vi "4Pi Astigmatism Alignment.vi"(7 "Calling VI Ref":refnum<vi>) -> ()   [LabVIEW 2016]
uses:
  <vilib>/Utility/miscctls.llb/LVPointTypeDef.ctl
  4Pi Astigmatism Alignment Type Defs/4Pi AA Notifier Type.ctl
  4Pi Astigmatism Alignment Type Defs/4Pi AA Actions.ctl
  <vilib>/vision/Image Controls.llb/IMAQ Image.ctl
  Hardware Configuration/Hardware Configuration Controls/Device Type.ctl
  Hardware Configuration/Hardware Configuration Controls/Device Function.ctl
  Device Library/Cameras/Hamamatsu/Orca Flash/Orca Flash Controls/Orca Flash Actions.ctl
  Device Library/Shutters/Shutter Controls/Shutter Actions.ctl
  Device Library/Stages/Stages Controls/Stage Actions.ctl
  <vilib>/Analysis/polynomials.llb/Polynomial Plot (Range).vi
  <vilib>/Analysis/NI_AALPro.lvlib
panel:
  out "Error":bool
  in  "Frame Accumulations":u16=1
  in  "Number of Steps":u16=10
  in  "Step Size (µm)":dbl=0.05
  in  "Scan and Align":bool
  in  "Scan Lower Obj":bool
  out "ROI Fit":dbl[][](graph)
  out "ROI Image":u16[][](graph)
  in  "Image Selection":i32(ring) items=["Quad 01", "Quad 02", "Quad 03", "Quad 04"]
  in  "Scan Upper Obj":bool
  in  "Quit":bool
  out "Scan Data":cluster{dbl[], dbl[]}[](graph)
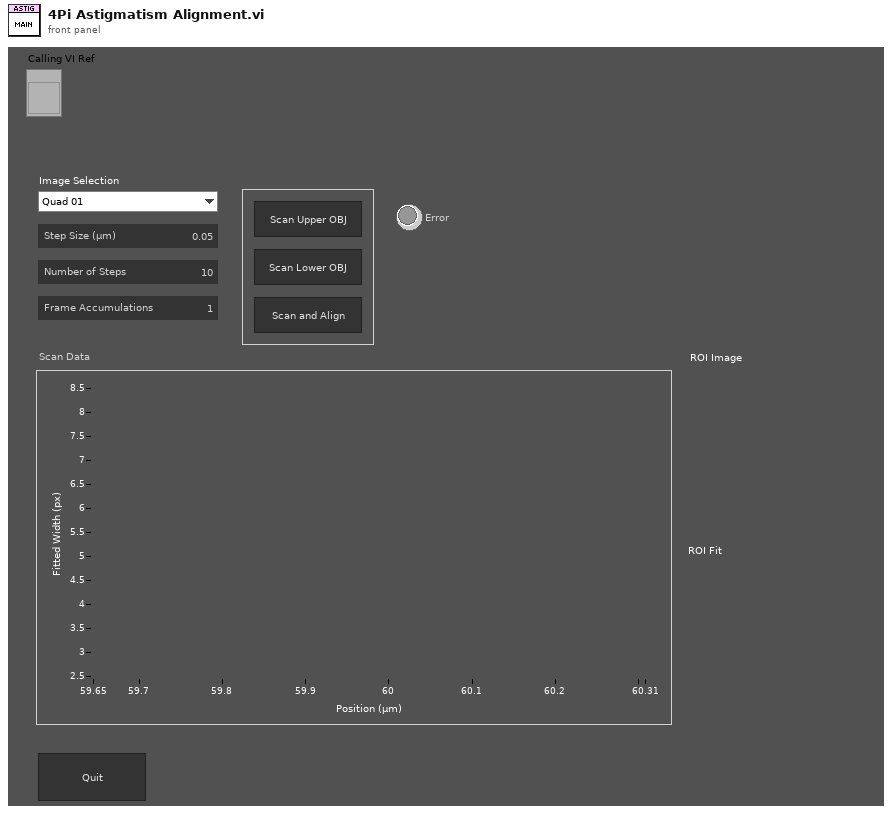
[diagram p1: front panel]
types:
  T1 = typedef "IMAQ Image.ctl" = refnum<image>
  T2 = typedef "4Pi AA Actions.ctl" = enum16{"Idle", "Scan Upper", "Scan Lower", "Scan and Align", "Open Shutter", "Close Shutter", "Set Z Start", "Get Image", "Plot Data", "Move Z Stage", "Fit Astig Curves", "Return Z Stage", "Switch", "Align OBJs", "Abort", "Quit"}
  T3 = typedef "4Pi AA Notifier Type.ctl" = cluster{"Actions":T2, "Scan Steps":u16, "Step Size (µm)":dbl, "Frame Accums":u16, "Image Ref":T1, "Initial Z Pos (µm)":dbl}
  T4 = enum16{"Always On", "Always Off", "Off While Running"}
  T5 = typedef "LVPointTypeDef.ctl" = cluster{"Horizontal":i16, "Vertical":i16}
  T6 = typedef "Device Function.ctl" = enum16{"Primary", "Secondary", "Overview", "Wide Field Drift Correction", "642 nm Excitation", "560 nm Excitation", "546 nm Excitation", "488 nm Excitation", "405 nm Excitation", "Objective Drift Correction", "Objective XY", "Objective Z", "Sample XY", "Sample Coarse Z", "Sample Z", "4Pi Lower", "4Pi Upper", "Adj Cavity", "Line Scanning", "Alert"}
  T7 = typedef "Device Type.ctl" = enum16{"AOTF", "Camera", "Deformable Mirror", "Laser", "Shutter", "Stage", "Waveform", "Email"}
  T8 = typedef "Orca Flash Actions.ctl" = enum16{"IDLE", "PREVIEW", "RECORD", "Record Settings", "SETPARAM", "GETPARAM", "SETROI", "GETROI", "PROGRESSIVE MODE", "AREA MODE", "STATUS", "QUIT"}
  T9 = typedef "Shutter Actions.ctl" = enum16{"Open", "Close", "Toggle", "Status", "Quit"}
  T10 = typedef "Stage Actions.ctl" = enum16{"Get Position", "MVR", "MOVE", "HALT", "ONTARGET", "ERROR", "REFERENCE", "INIT", "VELOCITY", "STATUS", "EXIT", "HOME", "ZEROPOS", "NANOPOS", "ANALOG", "QUIT"}
  T11 = enum32{"Invalid", "Standard", "Closed", "Hidden", "Minimized", "Maximized"}
  T12 = typedef "2D Gaussian - Best Fit Parameters.ctl" = cluster{"Amplitude":dbl, "X Position":dbl, "Y Position":dbl, "X Width":dbl, "Y Width":dbl, "Offset":dbl}
  T13 = typedef "LVRectTypeDef.ctl" = cluster{"Left":i16, "Top":i16, "Right":i16, "Bottom":i16}
  T14 = typedef "LVBoundsTypeDef.ctl" = cluster{"Width":u32, "Height":u32}
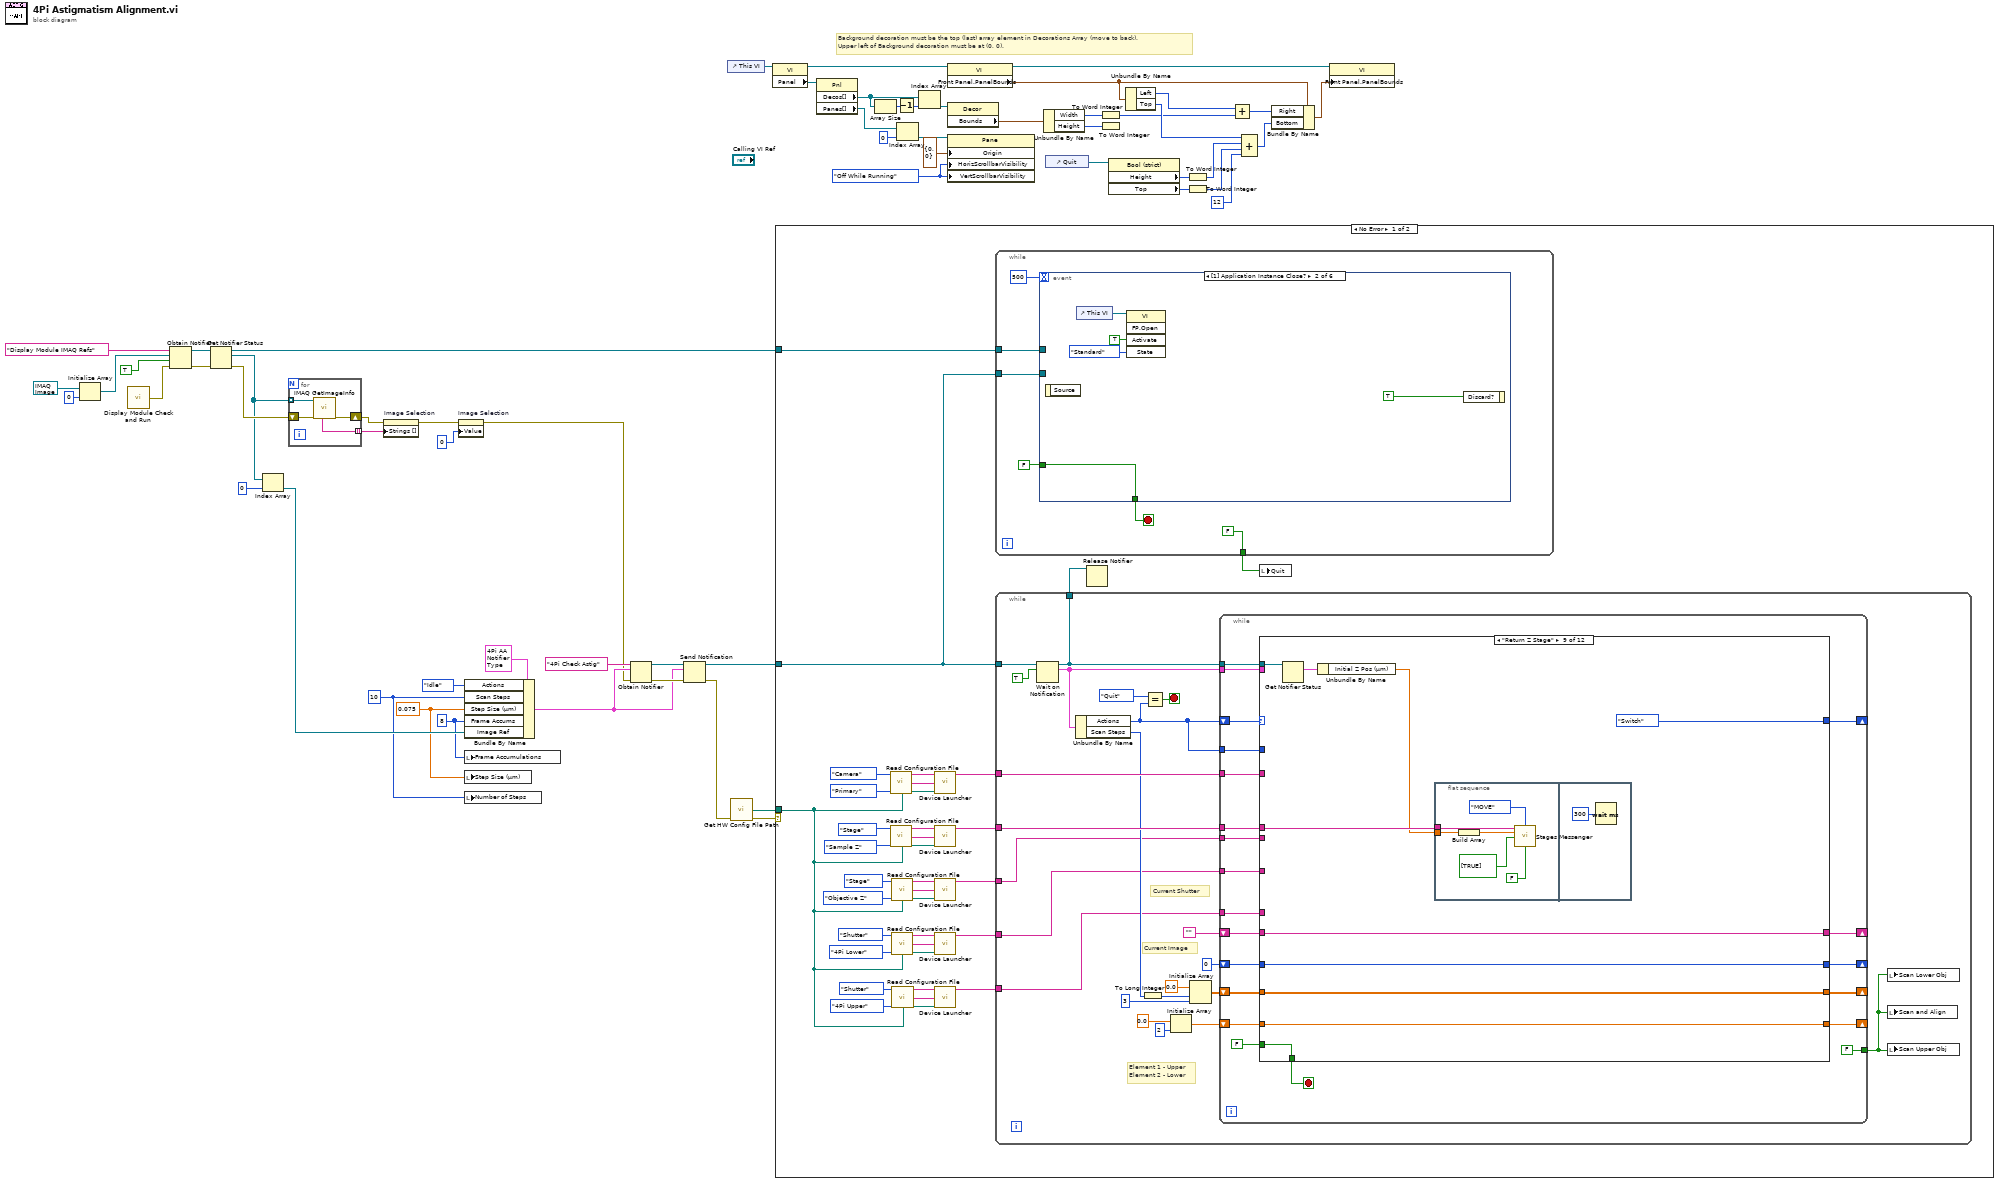
[diagram p0: block diagram]
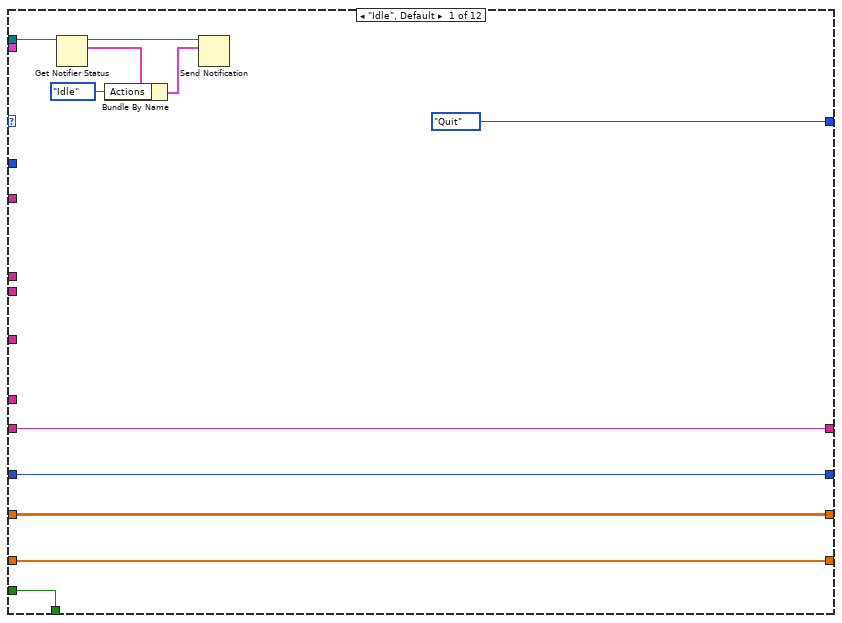
[diagram p2: hidden frame]
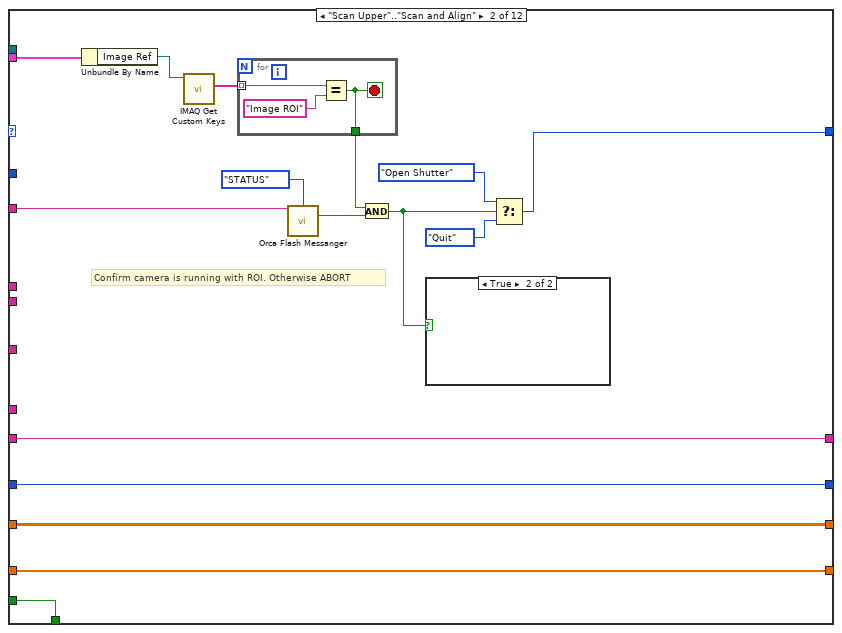
[diagram p3: hidden frame]
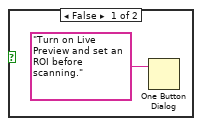
[diagram p4: hidden frame]
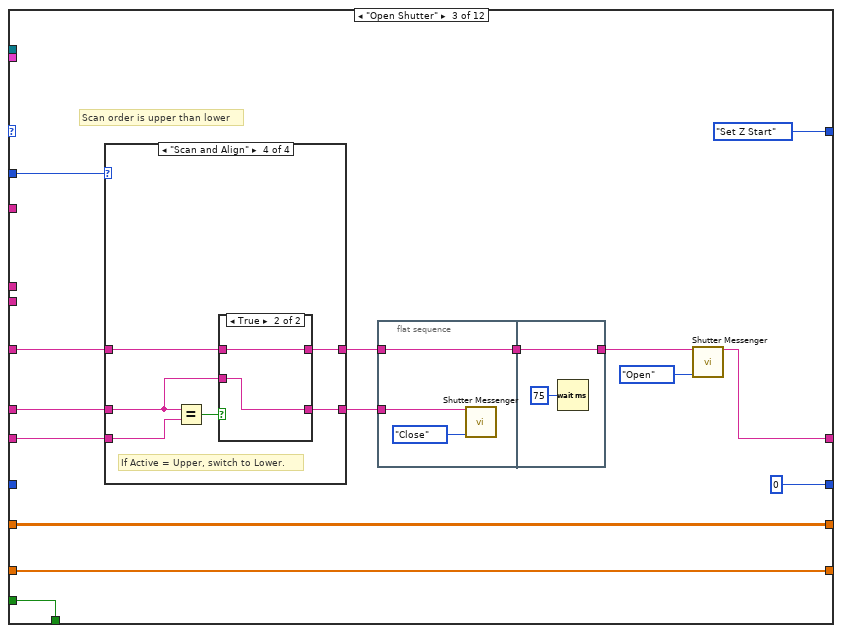
[diagram p5: hidden frame]
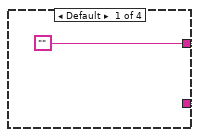
[diagram p6: hidden frame]
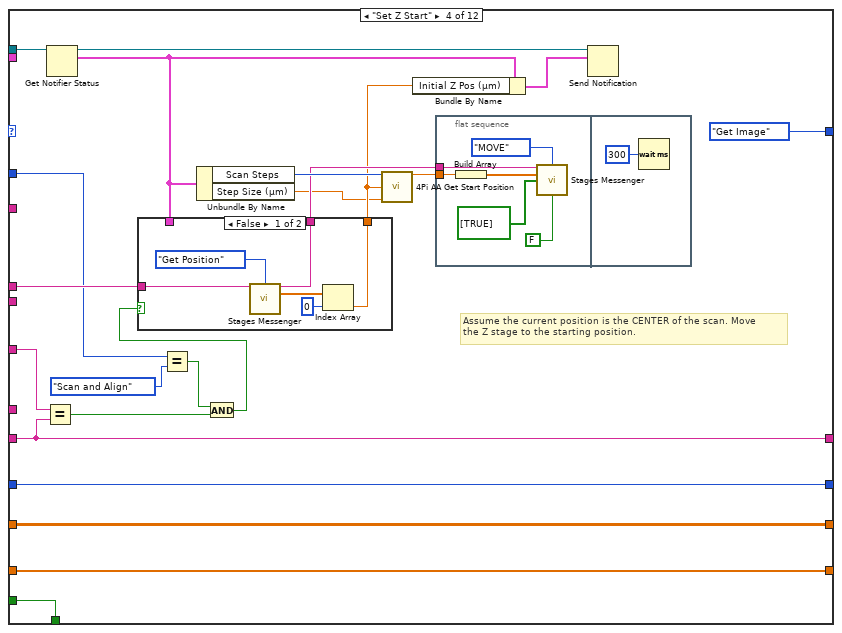
[diagram p10: hidden frame]
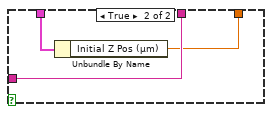
[diagram p11: hidden frame]
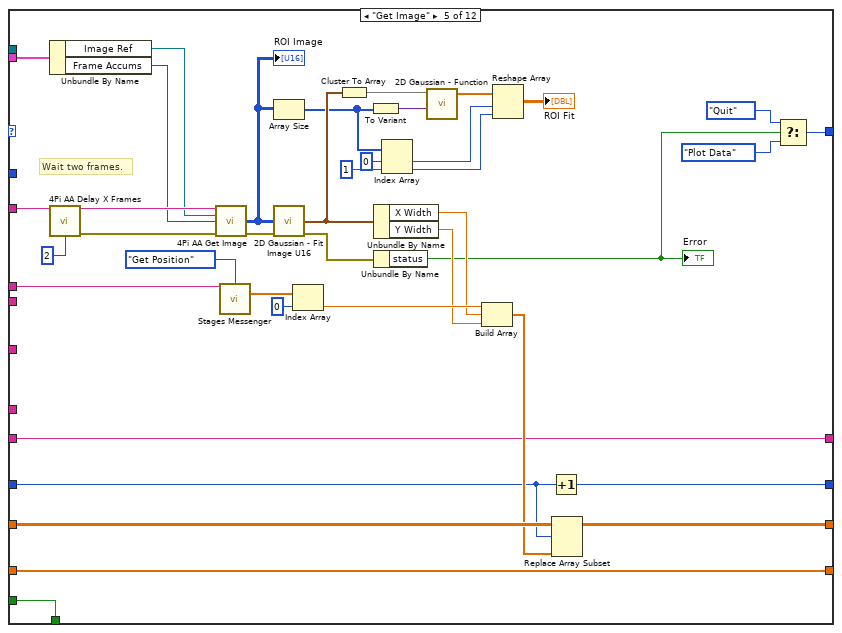
[diagram p12: hidden frame]
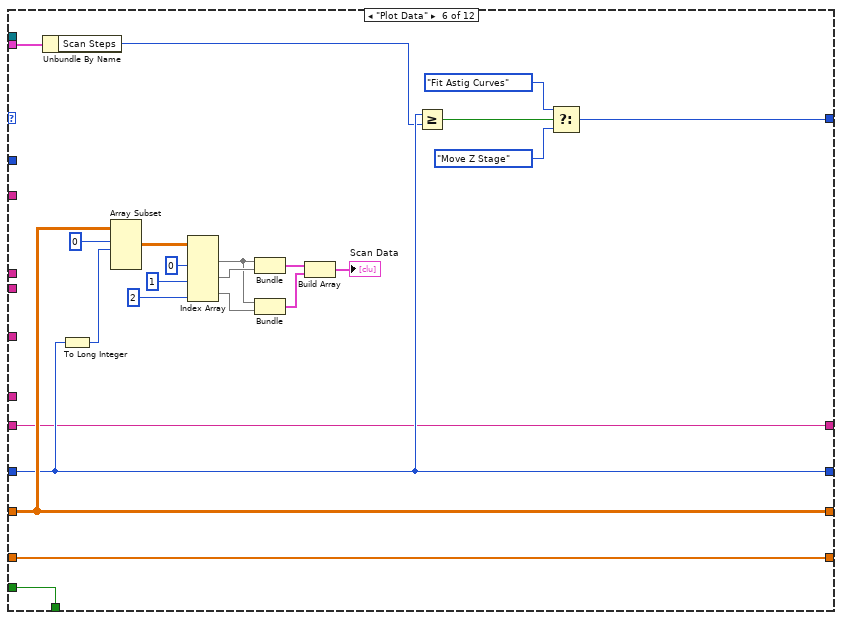
[diagram p13: hidden frame]
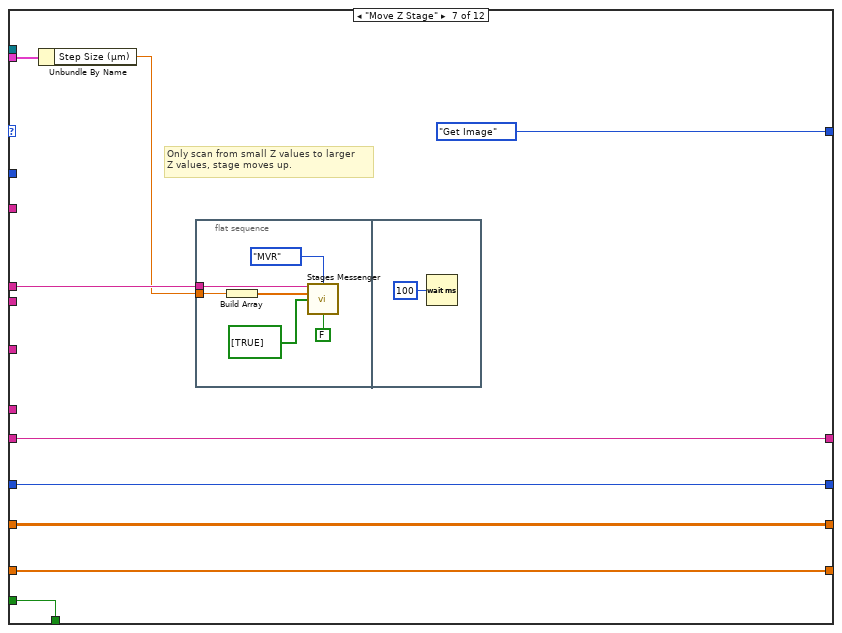
[diagram p14: hidden frame]
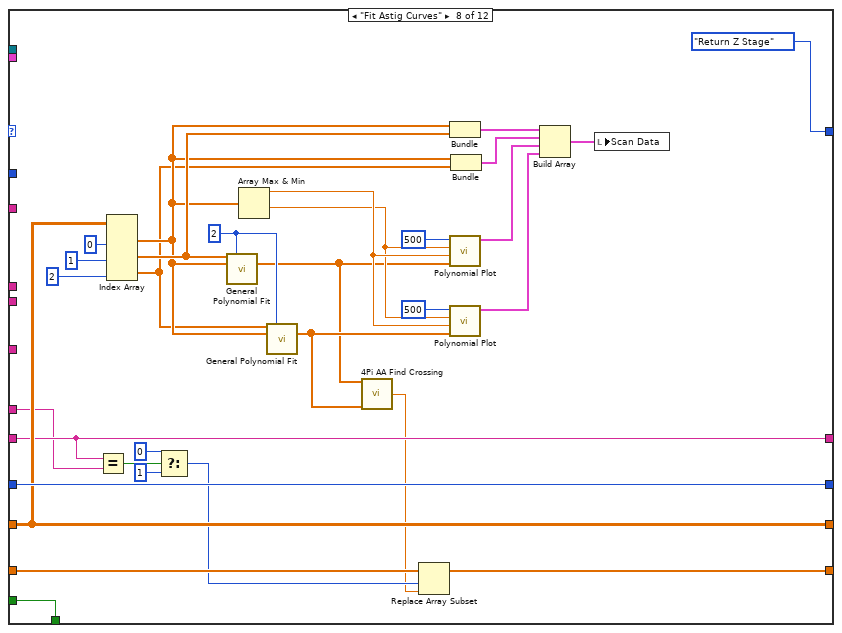
[diagram p15: hidden frame]
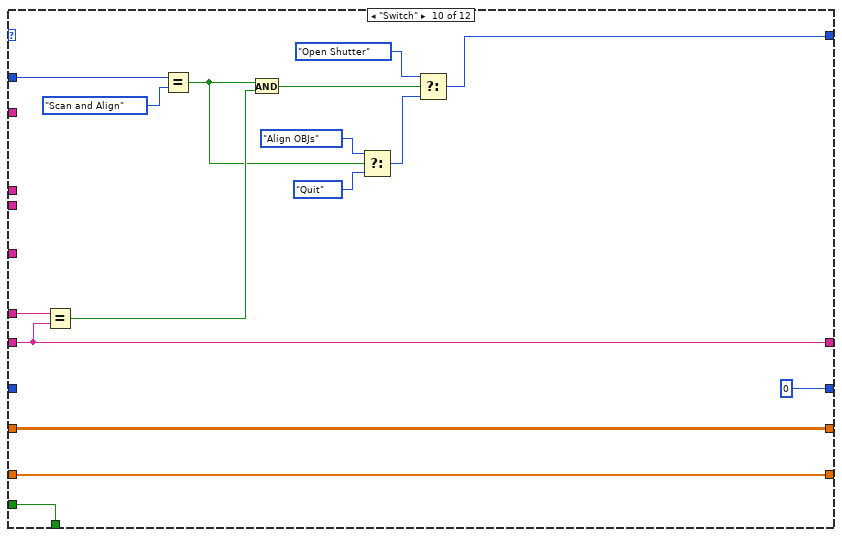
[diagram p16: hidden frame]
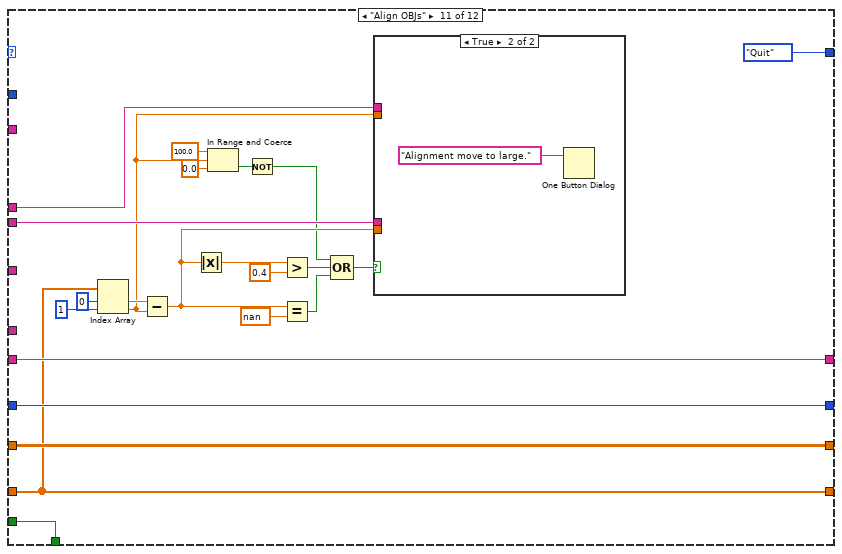
[diagram p17: hidden frame]
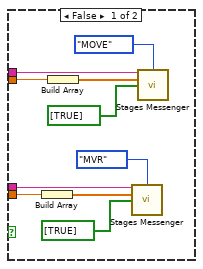
[diagram p18: hidden frame]
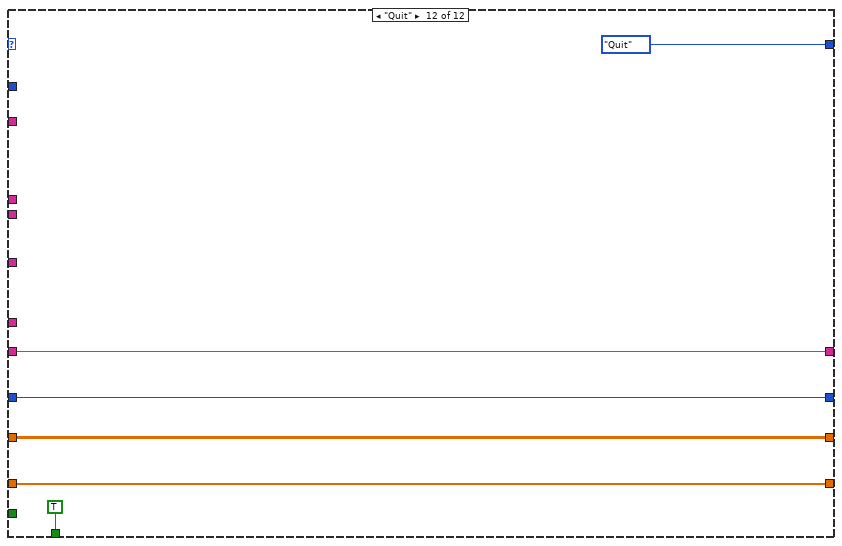
[diagram p19: hidden frame]
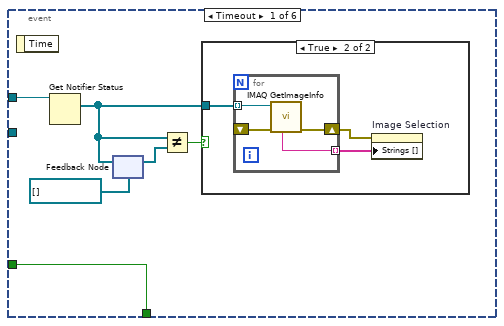
[diagram p20: hidden frame]
diagram:
  w3 = u16 8 ("Frame Accums")
  w2 = 0.075 ("Step Size (µm)")
  w1 = u16 10 ("Scan Steps")
  w41 = T4."Off While Running" ("Vertical Scrollbar Visibility")
  # "Background decoration must be the top (last) array element in Decorations Array (move to back).\nUpper left of Background decoration must be at (0, 0)."
  n1 = Initialize Array(T1 refnum ("New Image"), 0 ("dimension size")) -> (w17:T1[])
  n2 = call "Display Module Check and Run.vi"() -> ("Error"=w4:errorcluster)  [unwired: 15 in]
  n3 = Obtain Notifier(name (unnamed)="Display Module IMAQ Refs", notification data type=w17, create if not found? (T)=TRUE, error in (no error)=w4) -> (notifier out=w16:refnum<notifier>, error out=w15:errorcluster)  [unwired: 1 out]
  n4 = Get Notifier Status(notifier=w16, error in (no error)=w15) -> (notifier out=w14:refnum<notifier>, current notification=w8:T1[], error out=w13:errorcluster)  [unwired: 2 out]
  n5 = Index Array(array=w8, index=0) -> (element=w6:T1)
  n6 = for {
    tunnel: w8 -> [w64] mode=indexing
    shift-right: [w62] -> w11
    shift-left: w13 -> [w63]
    tunnel: [w61] -> w12 mode=indexing
    n7 = call "IMAQ GetImageInfo"("error in (no error)"=w63, "Image"=w64) -> ("error out"=w62:errorcluster, "Image Name"=w61:string)  [unwired: 2 in, 6 out]
  }
  n8 = property on="Image Selection" class="Ring (strict)"(error in=w11, "Strings []"=w12) -> (error out=w9:errorcluster)  [unwired: 1 in, 1 out]
  n9 = property on="Image Selection" class="Ring (strict)"(error in=w9, "Value"=0) -> (error out=w5:errorcluster)  [unwired: 1 in, 1 out]
  n10 = Bundle By Name(cluster=T3 {"Actions"=enum."Idle", "Scan Steps"=1, "Step Size (µm)"=0.1, "Frame Accums"=1, "Image Ref"=refnum, "Initial Z Pos (µm)"=0.0} ("Astig Test Data Type"), "Actions"=4Pi_AA_Actions."Idle", "Scan Steps"=w1, "Step Size (µm)"=w2, "Frame Accums"=w3, "Image Ref"=w6) -> (w22:T3)
  n11 = local write "Frame Accumulations"(w3) -> ()
  n12 = local write "Step Size (µm)"(w2) -> ()
  n13 = local write "Number of Steps"(w1) -> ()
  n14 = Obtain Notifier(name (unnamed)="4Pi Check Astig", notification data type=w22, error in (no error)=w5) -> (notifier out=w29:refnum<notifier>, error out=w28:errorcluster)  [unwired: 1 in, 1 out]
  n15 = Send Notification(notification=w22, notifier=w29, error in (no error)=w28) -> (notifier out=w25:refnum<notifier>, error out=w26:errorcluster)
  n16 = control-ref of="This VI"() -> (w33:refnum<vi>)
  n17 = call "Get HW Config File Path.vi"("Error"=w26) -> ("File Path"=w59:path, "Error"=w60:errorcluster)  [unwired: 13 in]
  n18 = property class="VI"(reference=w33) -> (reference out=w42:refnum<vi>, "Panel"=w34:refnum<vi>)  [unwired: 1 in, 1 out]
  n19 = case shown="No Error" w60 {
    tunnel: w59 -> [w66 _]
    tunnel: w25 -> [w87 _]
    tunnel: w14 -> [w84 _]
    frame No Error {
      n20 = call "Read Configuration File.vi"("Device Type"=Device_Type."Camera", "Device Function"=Device_Function."Primary", "Config File Path"=w66) -> ("Unique Notifier Name"=w97:string, "Device Ports/IDs/Channels"=w99:string[], "Device Engine Path"=w98:path)  [unwired: 9 in, 1 out]
      n21 = call "Read Configuration File.vi"("Device Type"=Device_Type."Stage", "Device Function"=Device_Function."Sample Z", "Config File Path"=w66) -> ("Unique Notifier Name"=w91:string, "Device Ports/IDs/Channels"=w89:string[], "Device Engine Path"=w90:path)  [unwired: 9 in, 1 out]
      n22 = call "Read Configuration File.vi"("Device Type"=Device_Type."Stage", "Device Function"=Device_Function."Objective Z", "Config File Path"=w66) -> ("Unique Notifier Name"=w74:string, "Device Ports/IDs/Channels"=w75:string[], "Device Engine Path"=w76:path)  [unwired: 9 in, 1 out]
      n23 = call "Read Configuration File.vi"("Device Type"=Device_Type."Shutter", "Device Function"=Device_Function."4Pi Lower", "Config File Path"=w66) -> ("Unique Notifier Name"=w83:string, "Device Ports/IDs/Channels"=w82:string[], "Device Engine Path"=w81:path)  [unwired: 9 in, 1 out]
      n24 = call "Read Configuration File.vi"("Device Type"=Device_Type."Shutter", "Device Function"=Device_Function."4Pi Upper", "Config File Path"=w66) -> ("Unique Notifier Name"=w67:string, "Device Ports/IDs/Channels"=w68:string[], "Device Engine Path"=w69:path)  [unwired: 9 in, 1 out]
      n25 = call "Device Launcher.vi"("Notifier Name"=w97, "Device Ports/IDs/Channels"=w99, "Device Engine Path"=w98) -> ("Notifier Name"=w85:string)  [unwired: 11 in, 1 out]
      n26 = call "Device Launcher.vi"("Notifier Name"=w91, "Device Ports/IDs/Channels"=w89, "Device Engine Path"=w90) -> ("Notifier Name"=w86:string)  [unwired: 11 in, 1 out]
      n27 = call "Device Launcher.vi"("Notifier Name"=w74, "Device Ports/IDs/Channels"=w75, "Device Engine Path"=w76) -> ("Notifier Name"=w73:string)  [unwired: 11 in, 1 out]
      n28 = call "Device Launcher.vi"("Notifier Name"=w83, "Device Ports/IDs/Channels"=w82, "Device Engine Path"=w81) -> ("Notifier Name"=w72:string)  [unwired: 11 in, 1 out]
      n29 = call "Device Launcher.vi"("Notifier Name"=w67, "Device Ports/IDs/Channels"=w68, "Device Engine Path"=w69) -> ("Notifier Name"=w65:string)  [unwired: 11 in, 1 out]
      n30 = while {
        tunnel: [FALSE] -> w94
        tunnel: w87 -> [w431]
        tunnel: w84 -> [w430]
        stop <- w433 stop-if-true
        n31 = event shown="[1] Application Instance Close?" {
          selector: _ -> [_ _ _ _ _ _]
          dyn-events: _ -> [_ _ _ _ _ _]
          timeout: 500 -> [_ _ _ _ _ _]
          tunnel: FALSE -> [w441 w452 w463 w472 w502 _]
          tunnel: [w441 w452 w463 w472 w502 w512] -> w433
          tunnel: w431 -> [_ _ w462 w471 w501 w507]
          tunnel: w430 -> [w440 _ w458 _ _ _]
          event Timeout {
            n32 = event-data() -> ()  [unwired: 1 in, 1 out]
            n33 = Get Notifier Status(notifier=w440) -> (current notification=w436:T1[])  [unwired: 1 in, 4 out]
            n34 = feedback-in #1(w436) -> ()
            n35 = feedback #1(T1[] []) -> (w438:T1[])
            n36 = Not Equal?(x=w436, y=w438) -> (x != y?=w437:bool)
            n37 = case shown="True" w437 {
              tunnel: w436 -> [_ w442]
              frame False {
              }
              frame True {
                n38 = for {
                  tunnel: w442 -> [w448] mode=indexing
                  shift-right: [w446] -> w443
                  shift-left: _ -> [w447]
                  tunnel: [w445] -> w444 mode=indexing
                  n39 = call "IMAQ GetImageInfo"("error in (no error)"=w447, "Image"=w448) -> ("error out"=w446:errorcluster, "Image Name"=w445:string)  [unwired: 2 in, 6 out]
                }
                n40 = property on="Image Selection" class="Ring (strict)"(error in=w443, "Strings []"=w444) -> ()  [unwired: 1 in, 2 out]
              }
            }
          }
          event Application Instance Close? {
            n41 = event-data() -> ()  [unwired: 1 in, 1 out]
            n42 = control-ref of="This VI"() -> (w449:refnum<vi>)
            n43 = invoke class="VI" method="FP.Open"(reference=w449, "Activate"=TRUE ("Activate?"), "State"=T11."Standard") -> ()  [unwired: 2 in, 5 out]
            n44 = event-data("Discard?"=TRUE) -> ()  [unwired: 1 in, 1 out]
          }
          event "Image Selection": Value Change {
            n45 = event-data() -> ("NewVal"=w455:i32)  [unwired: 1 in]
            n46 = Get Notifier Status(notifier=w458) -> (current notification=w457:T1[])  [unwired: 1 in, 4 out]
            n47 = Index Array(array=w457, index=w455) -> (element=w456:T1)
            n48 = Get Notifier Status(notifier=w462) -> (notifier out=w461:refnum<notifier>, current notification=w460:T3)  [unwired: 1 in, 3 out]
            n49 = Bundle By Name(cluster=w460, "Image Ref"=w456, "Actions"=4Pi_AA_Actions."Idle") -> (w459:T3)
            n50 = Send Notification(notification=w459, notifier=w461) -> ()  [unwired: 1 in, 2 out]
          }
          event "Step Size (µm)", "Number of Steps", "Frame Accumulations": Value Change {
            n51 = event-data() -> ("CtlRef"=w470:refnum<vi>)  [unwired: 1 in]
            n52 = property class="DigNum"(reference=w470) -> ("Label.Text"=w469:string)  [unwired: 1 in, 2 out]
            n53 = Get Notifier Status(notifier=w471) -> (notifier out=w468:refnum<notifier>, current notification=w467:T3)  [unwired: 1 in, 3 out]
            n54 = case shown="\"Step Size (µm)\"" w469 {
              tunnel: w468 -> [w476 w481 w486 w491]
              tunnel: w467 -> [w475 w480 w485 w490]
              tunnel: [w476 w481 w486 w491] -> w466
              tunnel: [w474 w479 w484 w489] -> w465
              tunnel: 4Pi_AA_Actions."Idle" ("Actions") -> [w473 w478 w483 w488]
              frame Default {
                n55 = Bundle By Name(cluster=w475, "Actions"=w473) -> (w474:T3)
              }
              frame "Number of Steps" {
                n56 = Bundle By Name(cluster=w480, "Scan Steps"="Number of Steps", "Actions"=w478) -> (w479:T3)
              }
              frame "Frame Accumulations" {
                n57 = Bundle By Name(cluster=w485, "Frame Accums"="Frame Accumulations", "Actions"=w483) -> (w484:T3)
              }
              frame "Step Size (µm)" {
                n58 = Bundle By Name(cluster=w490, "Step Size (µm)"="Step Size (µm)", "Actions"=w488) -> (w489:T3)
              }
            }
            n59 = Send Notification(notification=w465, notifier=w466) -> ()  [unwired: 1 in, 2 out]
          }
          event "Scan Upper Obj", "Scan Lower Obj", "Scan and Align": Value Change {
            n60 = event-data() -> ("CtlRef"=w497:refnum<vi>, "NewVal"=w493:bool)  [unwired: 1 in]
            n61 = property class="Bool (strict)"(reference=w497) -> ("Label.Text"=w496:string)  [unwired: 1 in, 2 out]
            n62 = case shown="\"Scan and Align\"" w496 {
              tunnel: [4Pi_AA_Actions."Idle" ("Actions") 4Pi_AA_Actions."Scan Upper" ("Actions") 4Pi_AA_Actions."Scan Lower" ("Actions") 4Pi_AA_Actions."Scan and Align" ("Actions")] -> w495
              frame Default {
              }
              frame "Scan Upper Obj" {
              }
              frame "Scan Lower Obj" {
              }
              frame "Scan and Align" {
              }
            }
            n63 = Select(t=w495, s=w493, f=4Pi_AA_Actions."Abort" ("Actions")) -> (s? t:f=w494:T2)
            n64 = Get Notifier Status(notifier=w501) -> (notifier out=w500:refnum<notifier>, current notification=w499:T3)  [unwired: 1 in, 3 out]
            n65 = Bundle By Name(cluster=w499, "Actions"=w494) -> (w498:T3)
            n66 = Send Notification(notification=w498, notifier=w500) -> ()  [unwired: 1 in, 2 out]
          }
          event "Quit": Value Change {
            n67 = event-data() -> ("NewVal"=w512:bool)  [unwired: 1 in]
            n68 = Get Notifier Status(notifier=w507) -> (notifier out=w511:refnum<notifier>, current notification=w510:T3)  [unwired: 1 in, 3 out]
            n69 = Bundle By Name(cluster=w510, "Actions"=4Pi_AA_Actions."Quit") -> (w509:T3)
            n70 = Send Notification(notification=w509, notifier=w511) -> ()  [unwired: 1 in, 2 out]
          }
        }
      }
      n71 = while {
        tunnel: w87 -> [w122]
        tunnel: [w118] -> w88
        tunnel: w86 -> [w117]
        tunnel: w85 -> [w115]
        tunnel: w73 -> [w106]
        tunnel: w72 -> [w105]
        tunnel: w65 -> [w104]
        stop <- w120 stop-if-true
        # "Element 1 - Upper\nElement 2 - Lower"
        # "Current Image"
        # "Current Shutter"
        n72 = Wait on Notification(notifier=w122, ignore previous (F)=TRUE) -> (notifier out=w118:refnum<notifier>, notification=w119:T3)  [unwired: 2 in, 2 out]
        n73 = Unbundle By Name(w119) -> ("Actions"=w107:T2, "Scan Steps"=w113:u16)
        n74 = To Long Integer(number=w113) -> (32bit integer=w110:i32)
        n75 = Equal?(x=4Pi_AA_Actions."Quit" ("y"), y=w107) -> (x = y?=w120:bool)
        n76 = Initialize Array(0.0 ("element"), 2 ("dimension size")) -> (w100:dbl[])
        n77 = Initialize Array(0.0 ("element"), w110, 3 ("dimension size")) -> (w111:dbl[][])
        n78 = while {
          tunnel: w119 -> [w140]
          shift-right: [w137] -> _
          shift-left: w107 -> [w143]
          tunnel: w118 -> [w139]
          tunnel: w117 -> [w138]
          shift-right: [w135] -> _
          shift-left: u16 0 -> [w136]
          tunnel: w115 -> [w134]
          shift-right: [w132] -> _
          shift-left: w111 -> [w133]
          tunnel: [FALSE] -> w108
          tunnel: w107 -> [w130]
          tunnel: w106 -> [w129]
          tunnel: w105 -> [w128]
          tunnel: w104 -> [w127]
          shift-right: [w125] -> _
          shift-left: "" -> [w126]
          shift-right: [w123] -> _
          shift-left: w100 -> [w124]
          stop <- w141 stop-if-true
          n79 = case shown="\"Return Z Stage\"" w143 {
            tunnel: FALSE -> [w154 w170 w189 w229 w286 w309 w318 w356 w363 w389 w411 _]
            tunnel: [w154 w170 w189 w229 w286 w309 w318 w356 w363 w389 w411 TRUE] -> w141
            tunnel: w140 -> [_ w167 _ _ w282 w306 w314 _ _ _ _ _]
            tunnel: w139 -> [w153 _ _ w212 _ _ _ _ w361 _ _ _]
            tunnel: w138 -> [_ _ _ w230 w278 _ w316 _ w362 _ w398 _]
            tunnel: [4Pi_AA_Actions."Quit" ("y") w160 4Pi_AA_Actions."Set Z Start" ("y") 4Pi_AA_Actions."Get Image" ("y") w250 w301 4Pi_AA_Actions."Get Image" ("y") 4Pi_AA_Actions."Return Z Stage" ("y") 4Pi_AA_Actions."Switch" ("y") w379 4Pi_AA_Actions."Quit" ("y") 4Pi_AA_Actions."Quit" ("y")] -> w137
            tunnel: [w146 w159 u16 0 w226 w271 w305 w317 w355 w365 u16 0 w409 w428] -> w135
            tunnel: w136 -> [w146 w159 _ w226 w270 w305 w317 w355 w365 _ w409 w428]
            tunnel: w134 -> [_ w169 _ _ w285 _ _ _ _ _ _ _]
            tunnel: w133 -> [w147 w158 w188 w225 w274 w308 w312 w353 w364 w388 w410 w427]
            tunnel: [w147 w158 w188 w225 w273 w308 w312 w353 w364 w388 w410 w427] -> w132
            tunnel: w130 -> [_ _ w185 w216 _ _ _ _ _ w386 _ _]
            tunnel: w129 -> [_ _ _ _ _ _ _ _ _ _ w407 _]
            tunnel: w128 -> [_ _ w183 w218 _ _ _ _ _ _ _ _]
            tunnel: w127 -> [_ _ w184 _ _ _ _ w333 _ w384 _ _]
            tunnel: w126 -> [w145 w157 w182 w219 w258 w288 w311 w334 w358 w382 w408 w425]
            tunnel: [w145 w157 w181 w219 w258 w288 w311 w334 w358 w382 w408 w425] -> w125
            tunnel: w124 -> [w144 w156 w175 w220 w257 w287 w310 w329 w357 w374 w403 w424]
            tunnel: [w144 w156 w175 w220 w257 w287 w310 w328 w357 w374 w403 w424] -> w123
            frame "Idle", Default {
              n80 = Get Notifier Status(notifier=w153) -> (notifier out=w152:refnum<notifier>, current notification=w151:T3)  [unwired: 1 in, 3 out]
              n81 = Bundle By Name(cluster=w151, "Actions"=4Pi_AA_Actions."Idle") -> (w149:T3)
              n82 = Send Notification(notification=w149, notifier=w152) -> ()  [unwired: 1 in, 2 out]
            }
            frame "Scan Upper".."Scan and Align" {
              # "Confirm camera is running with ROI. Otherwise ABORT"
              n83 = Unbundle By Name(w167) -> ("Image Ref"=w165:T1)
              n84 = call "IMAQ Get Custom Keys"("Image"=w165) -> ("Keys"=w166:string[])  [unwired: 7 in, 3 out]
              n85 = for {
                tunnel: w166 -> [w174] mode=indexing
                tunnel: [w172] -> w163
                stop <- w172 stop-if-true
                n86 = Equal?(x=w174, y="Image ROI") -> (x = y?=w172:bool)
              }
              n87 = call "Orca Flash Messanger.vi"("Notifier Name"=w169, "Camera Actions"=Orca_Flash_Actions."STATUS") -> ("Running?"=w164:bool)  [unwired: 9 in, 4 out]
              n88 = And(x=w163, y=w164) -> (x .and. y?=w155:bool)
              n89 = case shown="True" w155 {
                frame False {
                  n90 = One Button Dialog(message="Turn on Live Preview and set an ROI before scanning.") -> ()  [unwired: 1 in, 1 out]
                }
                frame True {
                }
              }
              n91 = Select(t=4Pi_AA_Actions."Open Shutter" ("y"), s=w155, f=4Pi_AA_Actions."Quit") -> (s? t:f=w160:T2)
            }
            frame "Open Shutter" {
              # "Scan order is upper than lower"
              n92 = case shown="\"Scan and Align\"" w185 {
                tunnel: w184 -> [_ w197 w198 w201]
                tunnel: w183 -> [_ w196 w199 w203]
                tunnel: [w195 w197 w199 w202] -> w179
                tunnel: w182 -> [_ _ _ w205]
                tunnel: [w195 w196 w198 w200] -> w176
                frame Default {
                  w195 = ""
                }
                frame "Scan Upper" {
                }
                frame "Scan Lower" {
                }
                frame "Scan and Align" {
                  # "If Active = Upper, switch to Lower."
                  n93 = Equal?(x=w201, y=w205) -> (x = y?=w204:bool)
                  n94 = case shown="True" w204 {
                    tunnel: w203 -> [w206 w209]
                    tunnel: [w207 w209] -> w202
                    tunnel: w201 -> [w207 w208]
                    tunnel: [w206 w208] -> w200
                    frame False {
                    }
                    frame True {
                    }
                  }
                }
              }
              n95 = flat-sequence {
                tunnel: w179 -> [w192]
                tunnel: [w192] -> w177
                tunnel: w176 -> [w190]
                tunnel: [w194] -> w178
                tunnel: w177 -> [w194]
                frame #0 {
                  n96 = call "Shutter Messenger.vi"("Notifier Name"=w190, "Action"=Shutter_Actions."Close") -> ()  [unwired: 12 in, 2 out]
                }
                frame #1 {
                  n97 = Wait (ms)(milliseconds to wait=u32 75) -> ()  [unwired: 1 out]
                }
              }
              n98 = call "Shutter Messenger.vi"("Notifier Name"=w178, "Action"=Shutter_Actions."Open") -> ("Notifier Name Dup"=w181:string)  [unwired: 12 in, 1 out]
            }
            frame "Set Z Start" {
              # "Assume the current position is the CENTER of the scan. Move\nthe Z stage to the starting position."
              n99 = Equal?(x=w218, y=w219) -> (x = y?=w217:bool)
              n100 = Get Notifier Status(notifier=w212) -> (notifier out=w211:refnum<notifier>, current notification=w210:T3)  [unwired: 1 in, 3 out]
              n101 = Equal?(x=w216, y=4Pi_AA_Actions."Scan and Align") -> (x = y?=w214:bool)
              n102 = Unbundle By Name(w210) -> ("Scan Steps"=w231:u16, "Step Size (µm)"=w221:dbl)
              n103 = And(x=w214, y=w217) -> (x .and. y?=w213:bool)
              n104 = case shown="False" w213 {
                tunnel: w230 -> [w237 w240]
                tunnel: [w233 w240] -> w228
                tunnel: [w232 w238] -> w223
                tunnel: w210 -> [_ w239]
                frame False {
                  n105 = call "Stages Messenger.vi"("Stage Notifier Name"=w237, "Actions"=Stage_Actions."Get Position") -> ("Stage Notifier Name (Dup)"=w233:string, "Positions"=w235:dbl[])  [unwired: 10 in, 2 out]
                  n106 = Index Array(array=w235, index=0) -> (element=w232:dbl)
                }
                frame True {
                  n107 = Unbundle By Name(w239) -> ("Initial Z Pos (µm)"=w238:dbl)
                }
              }
              n108 = call "4Pi AA Get Start Position.vi"("Number of Steps"=w231, "Center Value"=w223, "Step Size"=w221) -> ("Starting Value"=w222:dbl)  [unwired: 11 in, 1 out]
              n109 = Bundle By Name(cluster=w210, "Initial Z Pos (µm)"=w223) -> (w224:T3)
              n110 = flat-sequence {
                tunnel: w228 -> [w246]
                tunnel: w222 -> [w245]
                frame #0 {
                  n111 = Build Array(w245) -> (w243:dbl[])
                  n112 = call "Stages Messenger.vi"("Stage Notifier Name"=w246, "Actions"=Stage_Actions."MOVE", "Setpoint"=w243, "Axis"=bool[] [TRUE], "Exit While Busy?"=FALSE) -> ()  [unwired: 7 in, 4 out]
                }
                frame #1 {
                  n113 = Wait (ms)(milliseconds to wait=u32 300) -> ()  [unwired: 1 out]
                }
              }
              n114 = Send Notification(notification=w224, notifier=w211) -> ()  [unwired: 1 in, 2 out]
            }
            frame "Get Image" {
              # "Wait two frames."
              n115 = Unbundle By Name(w282) -> ("Image Ref"=w256:T1, "Frame Accums"=w255:u16)
              n116 = call "4Pi AA Delay X Frames.vi"("Camera Notifier Name"=w285, "Wait No. (1)"=u32 2) -> ("Camera Notifier Name (Dup)"=w283:string, "Error Out"=w254:errorcluster)  [unwired: 12 in]
              n117 = call "4Pi AA Get Image.vi"("Camera Notifier Name"=w283, "Image Ref"=w256, "Frame Accums."=w255, "Error In"=w254) -> ("Image Out"=w269:u16[][], "Error Out"=w253:errorcluster)  [unwired: 10 in]
              "ROI Image" <- w269
              n118 = call "Stages Messenger.vi"("Stage Notifier Name"=w278, "Actions"=Stage_Actions."Get Position") -> ("Positions"=w280:dbl[])  [unwired: 10 in, 3 out]
              n119 = Array Size(array=w269) -> (size(s)=w264:i32[])
              n120 = call "2D Gaussian - Fit Image U16.vi"("Image In (U16)"=w269, "Error In"=w253) -> ("Best Fit Params"=w267:T12, "Error Out"=w252:errorcluster)  [unwired: 12 in]
              n121 = Index Array(array=w280, index=0) -> (element=w277:dbl)
              n122 = Cluster To Array(cluster=w267) -> (array=w266:dbl[])
              n123 = To Variant(anything=w264) -> (Variant=w268:variant)
              n124 = Unbundle By Name(w267) -> ("X Width"=w275:dbl, "Y Width"=w276:dbl)
              n125 = Unbundle By Name(w252) -> ("status"=w248:bool)
              "Error" <- w248
              n126 = Index Array(array=w264, index #1=0 ("index"), index #2=1 ("index")) -> (element #1=w261:i32, element #2=w260:i32)
              n127 = call "2D Gaussian - Function.vi"("data"=w268, "a"=w266) -> ("f(X,a)"=w265:dbl[])  [unwired: 2 in, 2 out]
              n128 = Build Array(w277, w275, w276) -> (w272:dbl[])
              n129 = Reshape Array(w265, w261, w260) -> (→"ROI Fit":dbl[][])
              n130 = Increment(x=w270) -> (x+1=w271:u16)
              n131 = Replace Array Subset(array=w274, new element=w272, index (row)=w270) -> (w273:dbl[][])  [unwired: 1 in]
              n132 = Select(t=4Pi_AA_Actions."Quit", s=w248, f=4Pi_AA_Actions."Plot Data" ("y")) -> (s? t:f=w250:T2)
            }
            frame "Plot Data" {
              n133 = Unbundle By Name(w306) -> ("Scan Steps"=w304:u16)
              n134 = To Long Integer(number=w305) -> (32bit integer=w289:i32)
              n135 = Array Subset(array=w308, index (row)=0 ("index"), length (row)=w289) -> (w299:dbl[][])  [unwired: 2 in]
              n136 = Index Array(array=w299, index (col) #1=0 ("disabled index (col)"), index (col) #2=1 ("index (col)"), index (col) #3=2 ("index (col)")) -> (element #1=w293:dbl[], element #2=w295:dbl[], element #3=w294:dbl[])  [unwired: 3 in]
              n137 = Bundle(w293, w295) -> (w292:cluster{dbl[], dbl[]})  [unwired: 1 in]
              n138 = Bundle(w293, w294) -> (w291:cluster{dbl[], dbl[]})  [unwired: 1 in]
              n139 = Build Array(w292, w291) -> (→"Scan Data":cluster{dbl[], dbl[]}[])
              n140 = Greater Or Equal?(x=w305, y=w304) -> (x >= y?=w303:bool)
              n141 = Select(t=4Pi_AA_Actions."Fit Astig Curves" ("y"), s=w303, f=4Pi_AA_Actions."Move Z Stage" ("y")) -> (s? t:f=w301:T2)
            }
            frame "Move Z Stage" {
              # "Only scan from small Z values to larger\nZ values, stage moves up."
              n142 = Unbundle By Name(w314) -> ("Step Size (µm)"=w313:dbl)
              n143 = flat-sequence {
                tunnel: w316 -> [w321]
                tunnel: w313 -> [w320]
                frame #0 {
                  n144 = Build Array(w320) -> (w323:dbl[])
                  n145 = call "Stages Messenger.vi"("Stage Notifier Name"=w321, "Actions"=Stage_Actions."MVR", "Setpoint"=w323, "Axis"=bool[] [TRUE], "Exit While Busy?"=FALSE) -> ()  [unwired: 7 in, 4 out]
                }
                frame #1 {
                  n146 = Wait (ms)(milliseconds to wait=u32 100) -> ()  [unwired: 1 out]
                }
              }
            }
            frame "Fit Astig Curves" {
              w349 = 2 ("polynomial order")
              n147 = Equal?(x=w334, y=w333) -> (x = y?=w332:bool)
              n148 = Index Array(array=w353, index (col) #1=0 ("disabled index (col)"), index (col) #2=1 ("index (col)"), index (col) #3=2 ("index (col)")) -> (element #1=w343:dbl[], element #2=w344:dbl[], element #3=w342:dbl[])  [unwired: 3 in]
              n149 = Select(t=0 ("disabled index (col)"), s=w332, f=1) -> (s? t:f=w327:i32)
              n150 = call <vilib>:"General Polynomial Fit.vi"("Y"=w344, "polynomial order"=w349, "X"=w343) -> ("Polynomial Coefficients"=w335:dbl[])  [unwired: 9 in, 3 out]
              n151 = Array Max & Min(array=w343) -> (max value=w346:dbl, min value=w345:dbl)  [unwired: 2 out]
              n152 = call <vilib>:"General Polynomial Fit.vi"("Y"=w342, "polynomial order"=w349, "X"=w343) -> ("Polynomial Coefficients"=w336:dbl[])  [unwired: 9 in, 3 out]
              n153 = call "4Pi AA Find Crossing.vi"("Fit Parameters 01"=w335, "Fit Parameters 02"=w336) -> ("X Crossing Position"=w326:dbl)  [unwired: 13 in]
              n154 = Replace Array Subset(array=w329, new element=w326, index=w327) -> (w328:dbl[])
              n155 = Bundle(w343, w344) -> (w341:cluster{dbl[], dbl[]})  [unwired: 1 in]
              n156 = call-poly <vilib>:"Polynomial Plot.vi"("P(x)"=w335, "end"=w346, "start"=w345, "samples"=500) -> ("polynomial plot"=w339:cluster{"Ramp Pattern":dbl[], "P(A)":dbl[]})  [unwired: 6 in, 1 out]
              n157 = call-poly <vilib>:"Polynomial Plot.vi"("P(x)"=w336, "end"=w346, "start"=w345, "samples"=500) -> ("polynomial plot"=w338:cluster{"Ramp Pattern":dbl[], "P(A)":dbl[]})  [unwired: 6 in, 1 out]
              n158 = Bundle(w343, w342) -> (w340:cluster{dbl[], dbl[]})  [unwired: 1 in]
              n159 = Build Array(w341, w340, w339, w338) -> (w337:cluster{"Ramp Pattern":dbl[], "P(A)":dbl[]}[])
              n160 = local write "Scan Data"(w337) -> ()
            }
            frame "Return Z Stage" {
              n161 = Get Notifier Status(notifier=w361) -> (current notification=w360:T3)  [unwired: 1 in, 4 out]
              n162 = Unbundle By Name(w360) -> ("Initial Z Pos (µm)"=w359:dbl)
              n163 = flat-sequence {
                tunnel: w362 -> [w370]
                tunnel: w359 -> [w369]
                frame #0 {
                  n164 = Build Array(w369) -> (w368:dbl[])
                  n165 = call "Stages Messenger.vi"("Stage Notifier Name"=w370, "Actions"=Stage_Actions."MOVE", "Setpoint"=w368, "Axis"=bool[] [TRUE], "Exit While Busy?"=FALSE) -> ()  [unwired: 7 in, 4 out]
                }
                frame #1 {
                  n166 = Wait (ms)(milliseconds to wait=u32 300) -> ()  [unwired: 1 out]
                }
              }
            }
            frame "Switch" {
              n167 = Equal?(x=w384, y=w382) -> (x = y?=w383:bool)
              n168 = Equal?(x=w386, y=4Pi_AA_Actions."Scan and Align") -> (x = y?=w378:bool)
              n169 = And(x=w378, y=w383) -> (x .and. y?=w381:bool)
              n170 = Select(t=4Pi_AA_Actions."Align OBJs" ("f"), s=w378, f=4Pi_AA_Actions."Quit") -> (s? t:f=w375:T2)
              n171 = Select(t=4Pi_AA_Actions."Open Shutter" ("y"), s=w381, f=w375) -> (s? t:f=w379:T2)
            }
            frame "Align OBJs" {
              n172 = Index Array(array=w403, index #1=0 ("index"), index #2=1 ("index")) -> (element #1=w400:dbl, element #2=w394:dbl)
              n173 = Subtract(x=w400, y=w394) -> (x-y=w399:dbl)
              n174 = Absolute Value(x=w399) -> (abs(x)=w404:dbl)
              n175 = In Range and Coerce(upper limit=100.0, x=w394, lower limit=0.0) -> (In Range?=w391:bool)  [unwired: 1 out]
              n176 = Not(x=w391) -> (.not. x?=w390:bool)
              n177 = Greater?(x=w404, y=0.4) -> (0:w396:bool)
              n178 = Equal?(x=w399, y=nan) -> (x = y?=w397:bool)
              n179 = Compound Arithmetic op=OR(w390, w396, w397) -> (w395:bool)
              n180 = case shown="True" w395 {
                tunnel: w407 -> [w422 _]
                tunnel: w399 -> [w418 _]
                tunnel: w394 -> [w414 _]
                tunnel: w398 -> [w413 _]
                frame False {
                  n181 = Build Array(w418) -> (w420:dbl[])
                  n182 = Build Array(w414) -> (w416:dbl[])
                  n183 = call "Stages Messenger.vi"("Stage Notifier Name"=w422, "Actions"=Stage_Actions."MVR", "Setpoint"=w420, "Axis"=bool[] [TRUE]) -> ()  [unwired: 8 in, 4 out]
                  n184 = call "Stages Messenger.vi"("Stage Notifier Name"=w413, "Actions"=Stage_Actions."MOVE", "Setpoint"=w416, "Axis"=bool[] [TRUE]) -> ()  [unwired: 8 in, 4 out]
                }
                frame True {
                  n185 = One Button Dialog(message="Alignment move to large.") -> ()  [unwired: 1 in, 1 out]
                }
              }
            }
            frame "Quit" {
            }
          }
        }
        n186 = local write "Scan Lower Obj"(w108) -> ()
        n187 = local write "Scan and Align"(w108) -> ()
        n188 = local write "Scan Upper Obj"(w108) -> ()
      }
      n189 = Release Notifier(notifier=w88) -> ()  [unwired: 2 in, 3 out]
      n190 = local write "Quit"(w94) -> ()
    }
    frame Error {
    }
  }
  n191 = property class="Pnl"(reference=w34) -> ("Decos[]"=w32:refnum<vi>[], "Panes[]"=w38:refnum<vi>[])  [unwired: 1 in, 2 out]
  n192 = Array Size(array=w32) -> (size(s)=w30:i32)
  n193 = Decrement(x=w30) -> (x-1=w31:i32)
  n194 = Index Array(array=w38, index=0) -> (element=w37:refnum<vi>)
  n195 = Index Array(array=w32, index=w31) -> (element=w40:refnum<vi>)
  n196 = property class="VI"(reference=w42) -> (reference out=w44:refnum<vi>, "Front Panel.PanelBounds"=w45:T13)  [unwired: 1 in, 1 out]
  n197 = property class="Decor"(reference=w40) -> ("Bounds"=w43:T14)  [unwired: 1 in, 2 out]
  n198 = property class="Pane"(reference=w37, "Origin"=T5 {"Horizontal"=0, "Vertical"=0}, "HorizScrollbarVisibility"=w41, "VertScrollbarVisibility"=w41) -> ()  [unwired: 1 in, 2 out]
  n199 = Unbundle By Name(w43) -> ("Width"=w48:u32, "Height"=w51:u32)
  n200 = control-ref of="Quit"() -> (w35:refnum<vi>)
  n201 = To Word Integer(number=w48) -> (16bit integer=w50:i16)
  n202 = To Word Integer(number=w51) -> ()  [unwired: 1 out]
  n203 = property class="Bool (strict)"(reference=w35) -> ("Height"=w53:u32, "Top"=w54:i32)  [unwired: 1 in, 2 out]
  n204 = Unbundle By Name(w45) -> ("Left"=w47:i16, "Top"=w58:i16)
  n205 = To Word Integer(number=w53) -> (16bit integer=w56:i16)
  n206 = To Word Integer(number=w54) -> (16bit integer=w57:i16)
  n207 = Add(x=w47, y=w50) -> (x+y=w49:i16)
  n208 = Compound Arithmetic op=ADD(w58, w56, w57, i16 12 ("y")) -> (w52:i16)
  n209 = Bundle By Name(cluster=w45, "Right"=w49, "Bottom"=w52) -> (w46:T13)
  n210 = property class="VI"(reference=w44, "Front Panel.PanelBounds"=w46) -> ()  [unwired: 1 in, 2 out]
